vi "Select_Profile - Copy.vi"(0 "Enum":T1=enum."DCW") -> (7 "selected path":path)   [LabVIEW 2021]
uses:
  Control/Ini.ctl
  test_type.ctl
panel:
  in  "Enum 2":T1
  in  "Select Button 2":bool
  out "selected path 2":path caption="selected path"
  in  "Select Button":bool
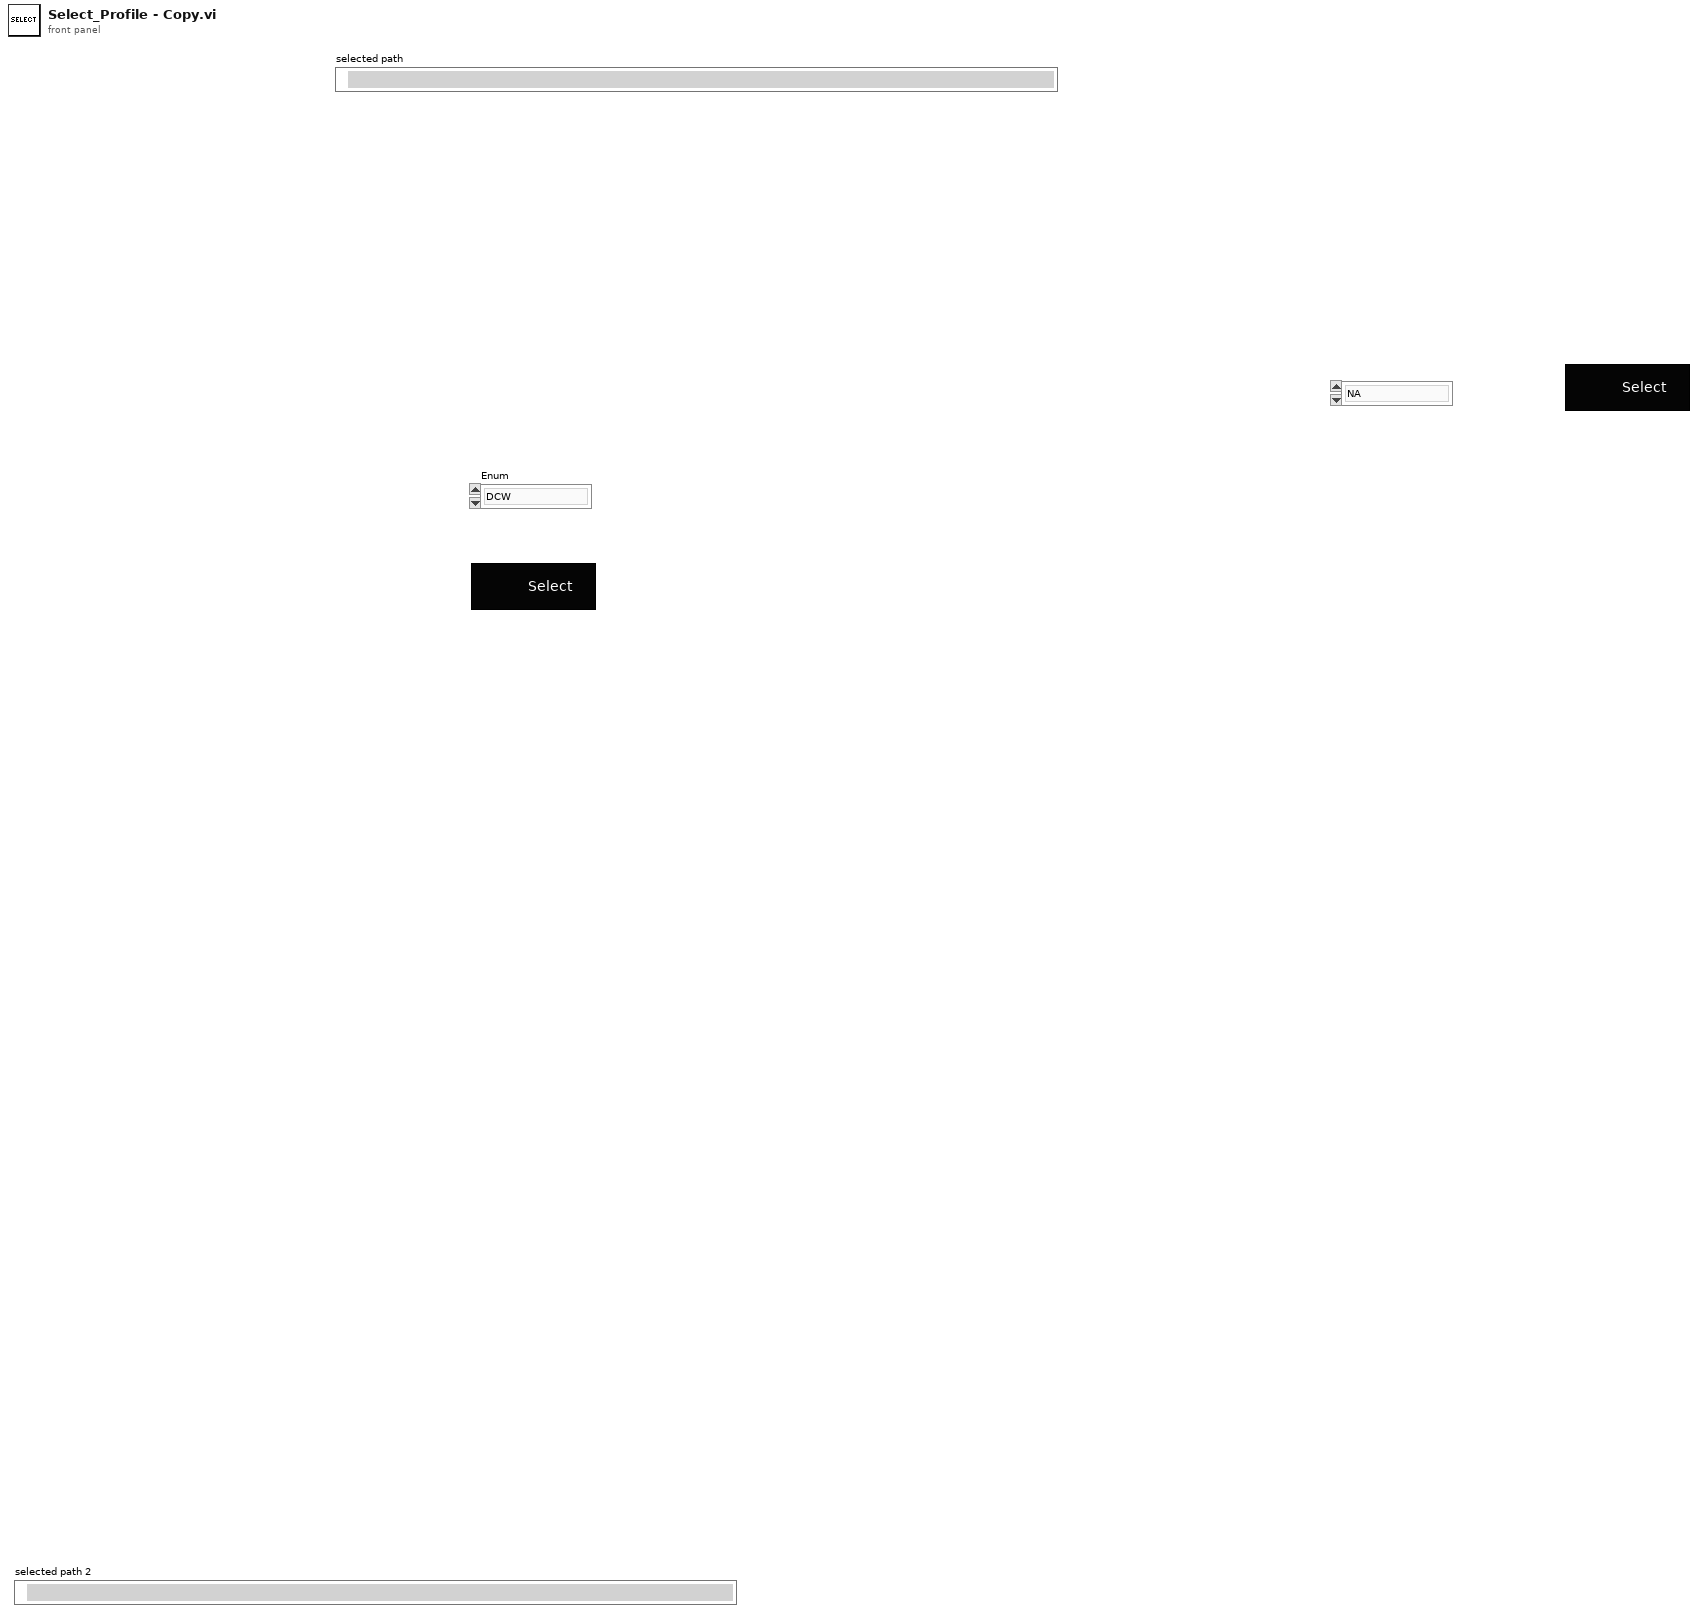
[diagram p1: front panel]
types:
  T1 = typedef "test_type.ctl" = enum16{"NA", "DCW", "ACW", "IR"}
  T2 = typedef "Ini.ctl" = enum16{"Write", "Read"}
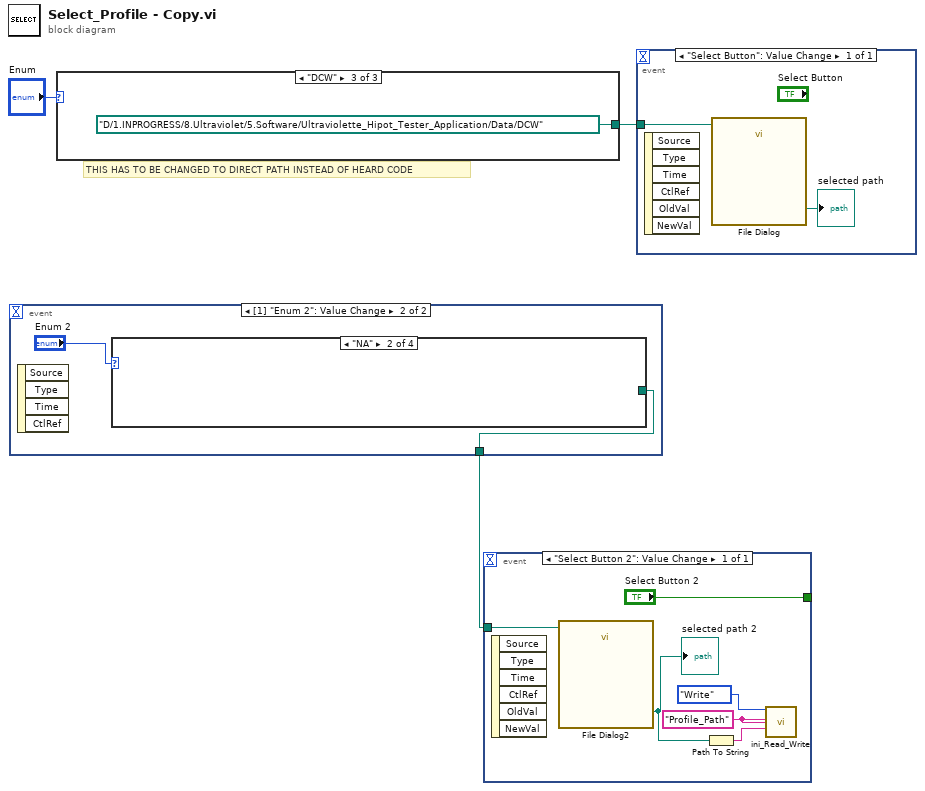
[diagram p0: block diagram]
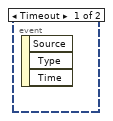
[diagram p2: hidden frame]
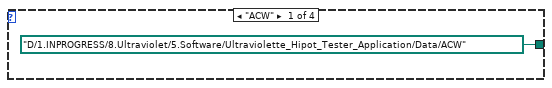
[diagram p3: hidden frame]
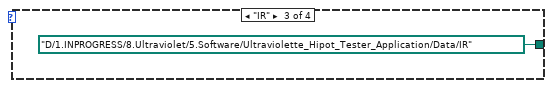
[diagram p4: hidden frame]
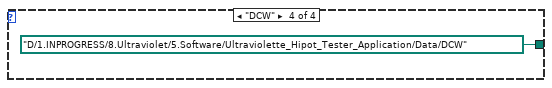
[diagram p5: hidden frame]
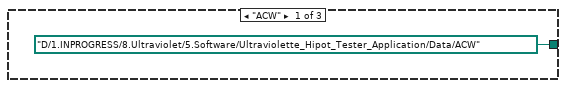
[diagram p6: hidden frame]
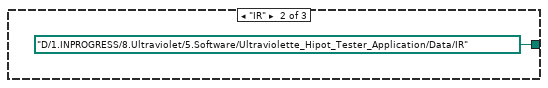
[diagram p7: hidden frame]
diagram:
  # "THIS HAS TO BE CHANGED TO DIRECT PATH INSTEAD OF HEARD CODE"
  n1 = event shown="[1] \"Enum 2\": Value Change" {
    selector: _ -> [_ _]
    dyn-events: _ -> [_ _]
    timeout: _ -> [_ _]
    tunnel: [_ w5] -> w1
    event Timeout {
      n2 = event-data() -> ()  [unwired: 1 in, 3 out]
    }
    event Value Change {
      n3 = event-data() -> ()  [unwired: 1 in, 4 out]
      n4 = case shown="\"NA\"" "Enum 2" {
        tunnel: [path "D:/1.INPROGRESS/8.Ultraviolet/5.Software/Ultraviolette_Hipot_Tester_Application/Data/ACW" ("start path") _ path "D:/1.INPROGRESS/8.Ultraviolet/5.Software/Ultraviolette_Hipot_Tester_Application/Data/IR" ("start path") path "D:/1.INPROGRESS/8.Ultraviolet/5.Software/Ultraviolette_Hipot_Tester_Application/Data/DCW" ("start path")] -> w5
        frame "ACW" {
        }
        frame "NA" {
        }
        frame "IR" {
        }
        frame "DCW" {
        }
      }
    }
  }
  n5 = case shown="\"DCW\"" "Enum" {
    tunnel: [path "D:/1.INPROGRESS/8.Ultraviolet/5.Software/Ultraviolette_Hipot_Tester_Application/Data/ACW" ("start path") path "D:/1.INPROGRESS/8.Ultraviolet/5.Software/Ultraviolette_Hipot_Tester_Application/Data/IR" ("start path") path "D:/1.INPROGRESS/8.Ultraviolet/5.Software/Ultraviolette_Hipot_Tester_Application/Data/DCW" ("start path")] -> w2
    frame "ACW" {
    }
    frame "IR" {
    }
    frame "DCW" {
    }
  }
  n6 = event shown="[0] \"Select Button 2\": Value Change" {
    selector: _ -> [_]
    dyn-events: _ -> [_]
    timeout: _ -> [_]
    tunnel: w1 -> [w17]
    tunnel: ["Select Button 2"] -> _
    event "Select Button 2": Value Change {
      w13 = "Profile_Path" ("Read Section")
      n7 = event-data() -> ()  [unwired: 1 in, 6 out]
      n8 = call "File Dialog2"("start path"=w17) -> ("selected path"=w12:path)  [unwired: 11 in, 3 out]
      "selected path 2" <- w12
      n9 = Path To String(path=w12) -> (string=w15:string)
      n10 = call "ini_Read_Write.vi"(0:Ini."Write", "Write Section"=w13, "Write key"=w13, "Write"=w15) -> ()  [unwired: 10 in, 2 out]
    }
  }
  n11 = event shown="[0] \"Select Button\": Value Change" {
    selector: _ -> [_]
    dyn-events: _ -> [_]
    timeout: _ -> [_]
    tunnel: w2 -> [w18]
    event "Select Button": Value Change {
      n12 = event-data() -> ()  [unwired: 1 in, 6 out]
      n13 = call "File Dialog"("start path"=w18) -> ("selected path"=→"selected path":path)  [unwired: 11 in, 3 out]
    }
  }
